vi "RDC-permittivity-Bilinear.vi"(8 "Salt Water":T1, 9 "DI-Water":T1, 10 "Open/Air":T1, 11 "Common Format":T1) -> (3 "Common Format out":T1)   [LabVIEW 2020, in "RDC-Reflection_Data_Computation.lvlib"]
doc: "Computes the permittivity of a Common Format cluster with the Bilinear method from the three standards Open/Air, DI water and salt water, solving a linear equation system per frequency."
uses:
  RDC-Reflection_Data_Computation.lvlib
  Reflector/RFH-common_data_format.ctl
  <vilib>/Analysis/7linalg.llb/Solve Complex Linear Equations (single right hand).vi
  <vilib>/Analysis/NI_AALPro.lvlib
  Reflector/RFH-Reflection_File_Handler.lvlib
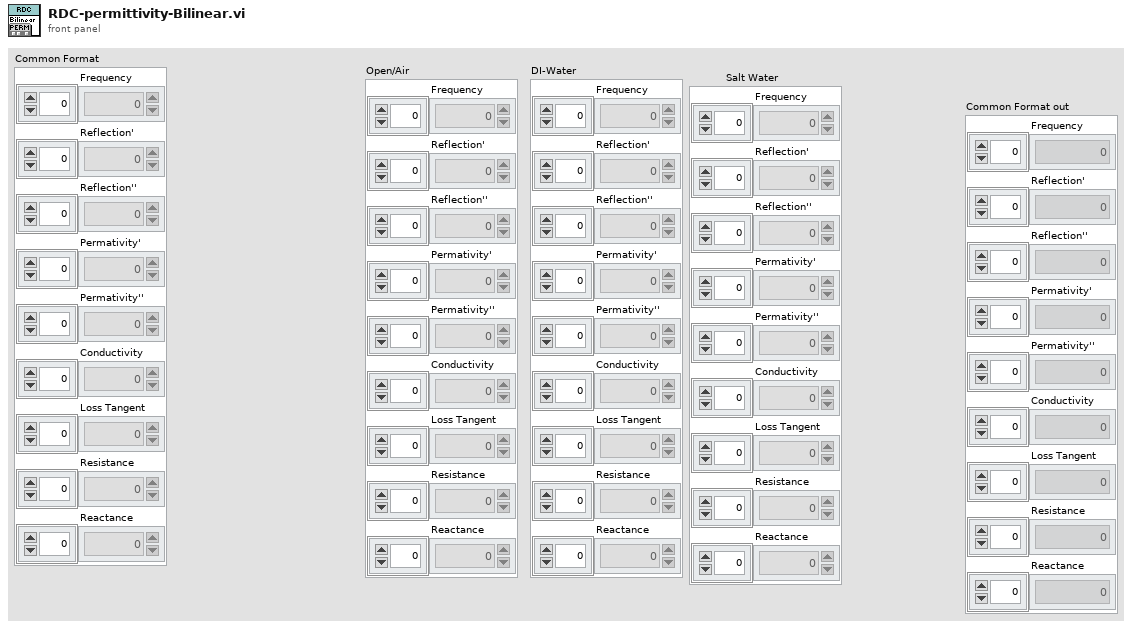
[diagram p1: front panel]
types:
  T1 = typedef "RFH-Reflection_File_Handler.lvlib/RFH-common_data_format.ctl" = cluster{"Frequency":dbl[], "Reflection'":dbl[], "Reflection''":dbl[], "Permativity'":dbl[], "Permativity''":dbl[], "Conductivity":dbl[], "Loss Tangent":dbl[], "Resistance":dbl[], "Reactance":dbl[]}
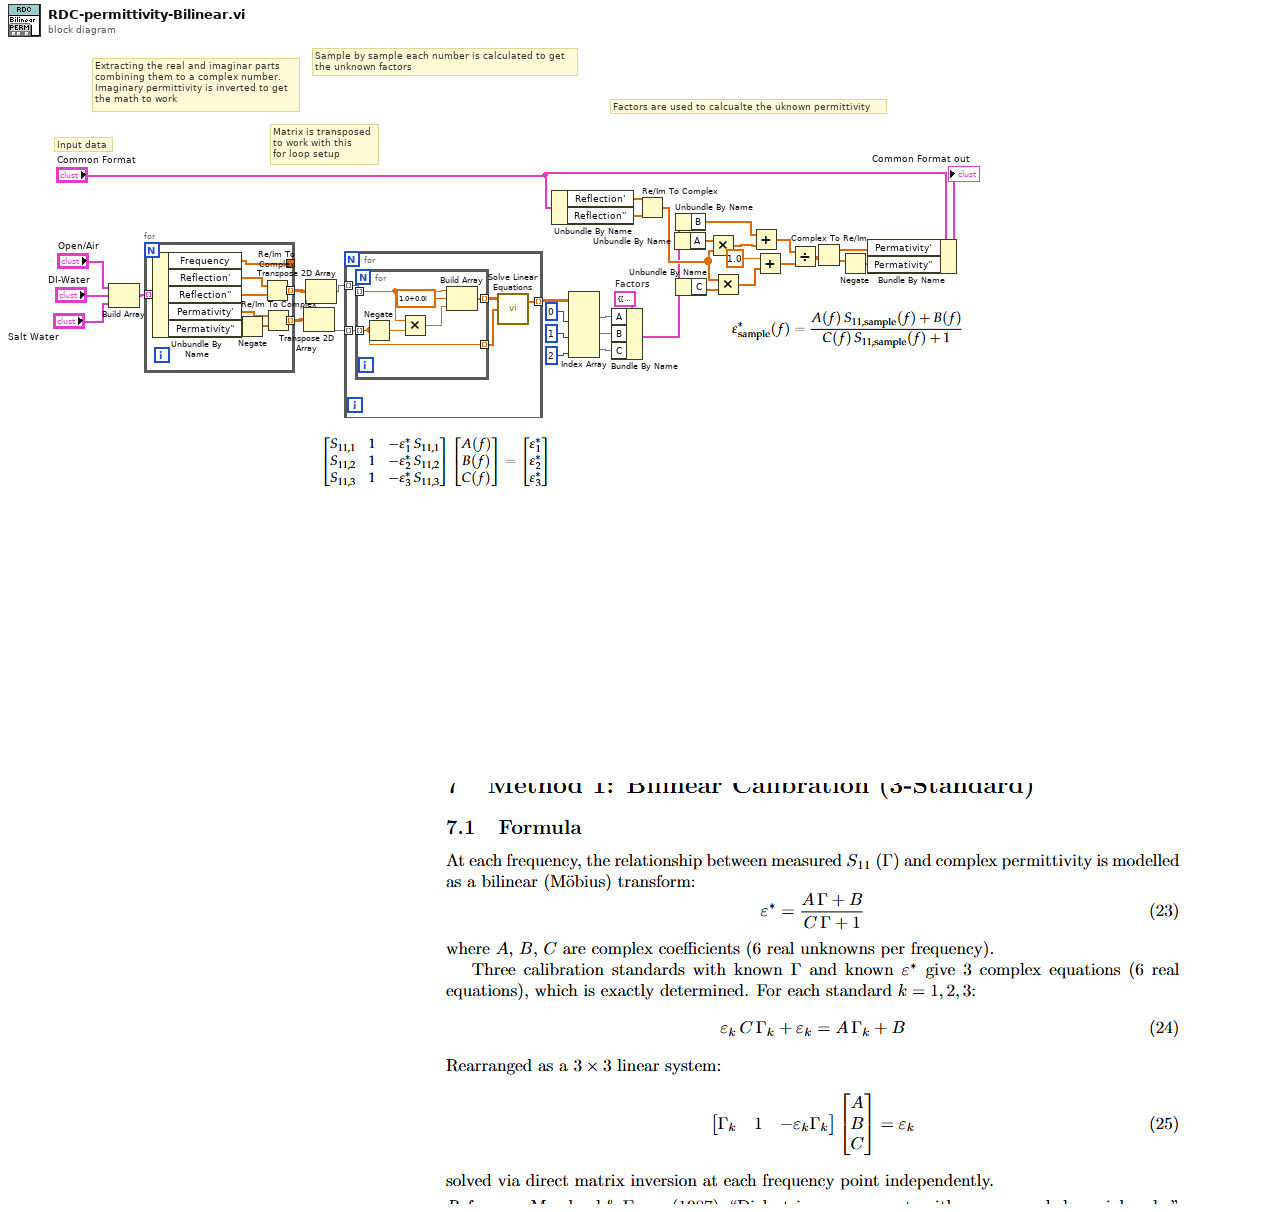
[diagram p0: block diagram]
diagram:
  w27 = cluster{"A":cdb[], "B":cdb[], "C":cdb[]} {"A"=[], "B"=[], "C"=[]}  # Factors
  # "Factors are used to calcualte the uknown permittivity"
  # "Sample by sample each number is calculated to get\nthe unknown factors"
  # "Matrix is transposed\nto work with this\nfor loop setup"
  # "Extracting the real and imaginar parts\ncombining them to a complex number.\nImaginary permittivity is inverted to get \nthe math to work"
  # "Input data"
  n1 = Build Array("Open/Air", "DI-Water", "Salt Water") -> (w34:T1[])
  n2 = for {
    tunnel: w34 -> [w43] mode=indexing
    tunnel: [w38] -> w23 mode=indexing
    tunnel: [w37] -> w22 mode=indexing
    tunnel: [w36] -> _
    n3 = Unbundle By Name(w43) -> ("Frequency"=w36:dbl[], "Reflection'"=w42:dbl[], "Reflection''"=w41:dbl[], "Permativity'"=w40:dbl[], "Permativity''"=w39:dbl[])
    n4 = Negate(x=w39) -> (-x=w35:dbl[])
    n5 = Re/Im To Complex(1:w41, 2:w42) -> (0:w38:cdb[])
    n6 = Re/Im To Complex(1:w35, 2:w40) -> (0:w37:cdb[])
  }
  n7 = Transpose 2D Array(2D array=w22) -> (transposed array=w32:cdb[][])
  n8 = Transpose 2D Array(2D array=w23) -> (transposed array=w33:cdb[][])
  n9 = for {
    tunnel: w33 -> [w47] mode=indexing
    tunnel: w32 -> [w48] mode=indexing
    tunnel: [w44] -> w31 mode=indexing
    n10 = for {
      tunnel: w48 -> [w53] mode=indexing
      tunnel: w47 -> [w50] mode=indexing
      tunnel: [w53] -> w45 mode=indexing
      tunnel: [w49] -> w46 mode=indexing
      n11 = Negate(x=w53) -> (-x=w54:cdb)
      n12 = Multiply(x=w50, y=w54) -> (x*y=w52:cdb)
      n13 = Build Array(w50, cdb 1.0+0.0i ("element"), w52) -> (w49:cdb[])
    }
    n14 = call-poly <vilib>:"Solve Linear Equations.vi"("Known Vector"=w45, "Input Matrix"=w46) -> ("Solution Vector"=w44:cdb[])  [unwired: 1 in, 1 out]
  }
  n15 = Unbundle By Name("Common Format") -> ("Reflection'"=w15:dbl[], "Reflection''"=w14:dbl[])
  n16 = Index Array(array=w31, index (col) #1=0 ("index (row)"), index (col) #2=1 ("index (row)"), index (col) #3=2 ("index (row)")) -> (element #1=w26:cdb[], element #2=w25:cdb[], element #3=w24:cdb[])  [unwired: 3 in]
  n17 = Bundle By Name(cluster=w27, "A"=w26, "B"=w25, "C"=w24) -> (w5:cluster{"A":cdb[], "B":cdb[], "C":cdb[]})
  n18 = Re/Im To Complex(1:w14, 2:w15) -> (0:w18:cdb[])
  n19 = Unbundle By Name(w5) -> ("A"=w4:cdb[])
  n20 = Unbundle By Name(w5) -> ("B"=w6:cdb[])
  n21 = Unbundle By Name(w5) -> ("C"=w7:cdb[])
  n22 = Multiply(x=w4, y=w18) -> (x*y=w20:cdb[])
  n23 = Multiply(x=w18, y=w7) -> (x*y=w17:cdb[])
  n24 = Add(x=w6, y=w20) -> (x+y=w19:cdb[])
  n25 = Add(x=1.0, y=w17) -> (x+y=w16:cdb[])
  n26 = Divide(x=w19, y=w16) -> (x/y=w12:cdb[])
  n27 = Complex To Re/Im(x + iy=w12) -> (x=w10:dbl[], y=w13:dbl[])
  n28 = Negate(x=w13) -> (-x=w11:dbl[])
  n29 = Bundle By Name(cluster="Common Format", "Permativity'"=w10, "Permativity''"=w11) -> (→"Common Format out":T1)
